vi "test_Basic Waveform Read and Write.vi"(8 "error in (no error)":errorcluster, 11 "DMA Channels Basic Testing in":refnum<class "FPGA Addon DMA Channels Basic System Tests.lvclass">) -> (0 "error out":errorcluster, 3 "DMA Channels Basic Testing out":refnum<class "FPGA Addon DMA Channels Basic System Tests.lvclass">)   [LabVIEW 2020, in "FPGA Addon DMA Channels Basic System Tests.lvclass"]
uses:
  FPGA Addon DMA Channels Basic System Tests.lvclass
  FPGA Addon Test Class/FPGA Addon Test Class.lvclass
panel:
  out "Waveform 2":waveform(dbl)(graph)
  out "Waveform 1":waveform(dbl)(graph)
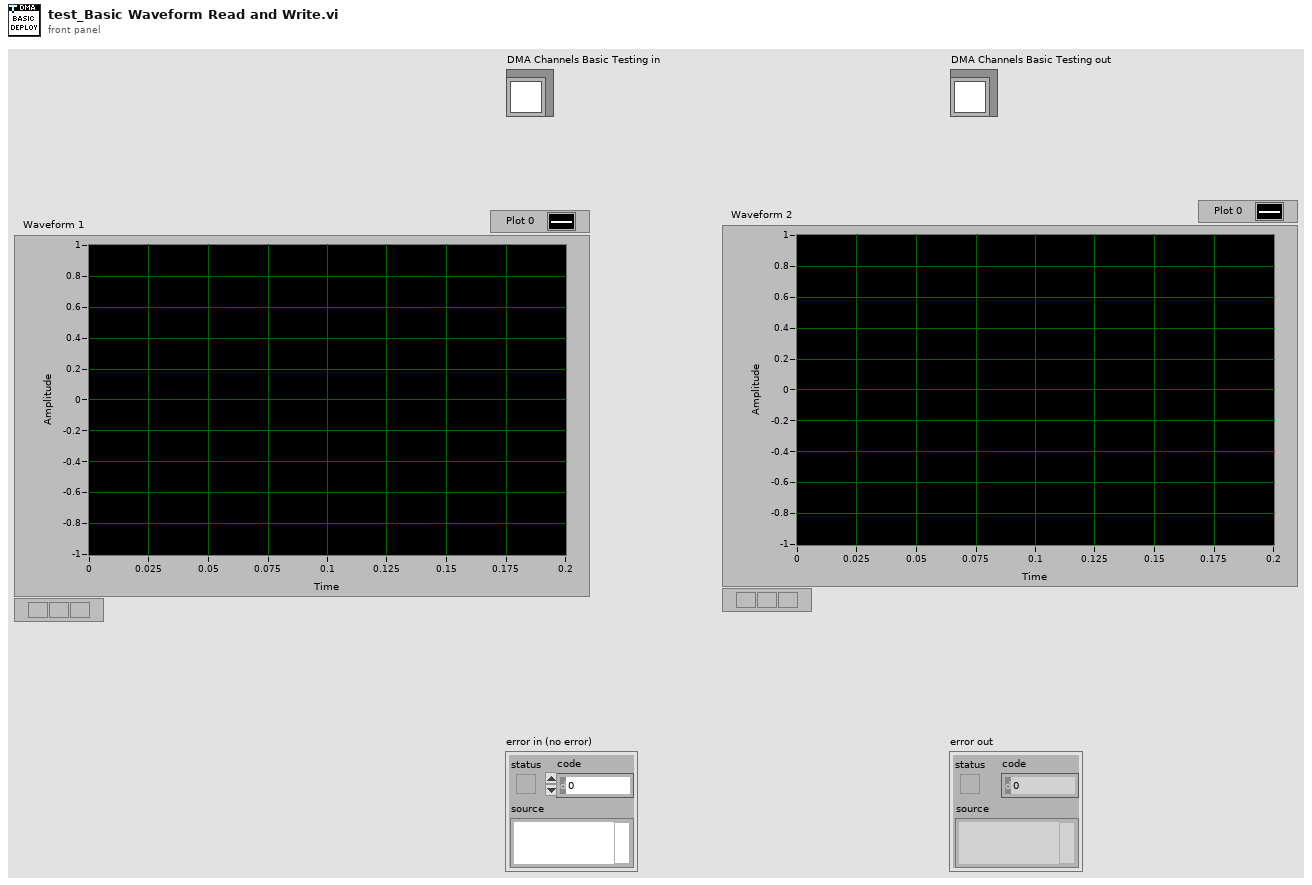
[diagram p1: front panel]
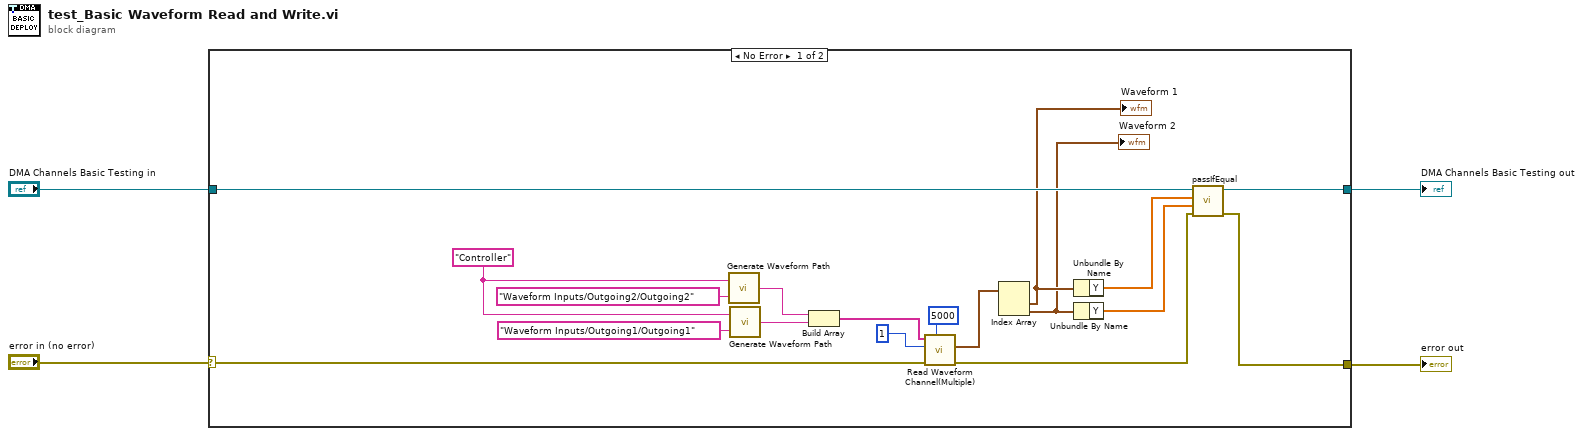
[diagram p0: block diagram]
diagram:
  n1 = case shown="No Error" "error in (no error)" {
    selector: "error in (no error)" -> [w17 w23]
    tunnel: "DMA Channels Basic Testing in" -> [w20 w24]
    tunnel: [w18 w24] -> w1
    tunnel: [w19 w23] -> w3
    frame No Error {
      w9 = "Controller" ("Target Name")
      n2 = call "Generate Waveform Path.vi"("Relative Waveform Path"="Waveform Inputs/Outgoing2/Outgoing2", "Target Name"=w9) -> ("Waveform Path Out"=w7:string)
      n3 = call "Generate Waveform Path.vi"("Relative Waveform Path"="Waveform Inputs/Outgoing1/Outgoing1", "Target Name"=w9) -> ("Waveform Path Out"=w6:string)
      n4 = Build Array(w7, w6) -> (w5:string[])
      n5 = call "Read Waveform Channel(Multiple).vi"("Timeout"=5000, "error in (no error)"=w17, "Number of Reads"=1, "Waveform Paths in"=w5) -> ("error out"=w14:errorcluster, "Waveform Data"=w15:waveform(dbl)[])  [unwired: 5 in, 1 out]
      n6 = Index Array(array=w15) -> (element #1=w13:waveform(dbl), element #2=w12:waveform(dbl))  [unwired: 2 in]
      "Waveform 1" <- w13
      "Waveform 2" <- w12
      n7 = Unbundle By Name(w13) -> ("Y"=w22:dbl[])
      n8 = Unbundle By Name(w12) -> ("Y"=w21:dbl[])
      n9 = call-dynamic "passIfEqual.vi"("error in (no error)"=w14, "y"=w21, "x"=w22, "TestCase in"=w20) -> ("error out"=w19:errorcluster, "TestCase out"=w18:refnum<class "FPGA Addon DMA Channels Basic System Tests.lvclass">)  [unwired: 6 in]
    }
    frame Error {
    }
  }
  "error out" <- w3
  "DMA Channels Basic Testing out" <- w1
